vi "Build Spec.vi"() -> ()   [LabVIEW 2020]
doc: "Builds a build specification of a project (scratch helper)"
panel:
  out "error out":errorcluster
  out "files":path[](array[path])
  in  "spec":string
  in  "project":path
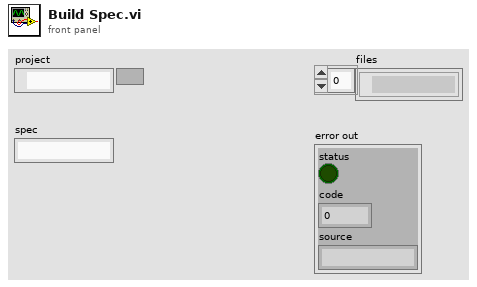
[diagram p1: front panel]
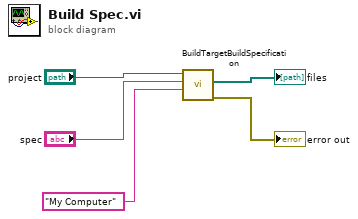
[diagram p0: block diagram]
diagram:
  n1 = call <vilib>:"BuildTargetBuildSpecification.vi"("Name of target (My Computer)"="My Computer", "Name of build specification (if empty: build all)"="spec", "Path to project"="project") -> ("error out"=→"error out":errorcluster, "Generated files"=→"files":path[])  [unwired: 7 in]
